vi "Render Read Pixels.vi"(6 "Pitch":i32 format="%.0x", 8 "error in":errorcluster, 9 "Format":u32 format="%.0x", 10 "Rectangle":T1, 11 "Renderer Pointer":u32 format="%.0x") -> (0 "error out":errorcluster, 2 "Pixels":i32[][](array[numeric]), 3 "Return":i32)   [LabVIEW 2021, in "LibSDL2.lvlib"]
uses:
  LibSDL2.lvlib
  DLL/SDL2.dll
  Controls/Rectangle.ctl
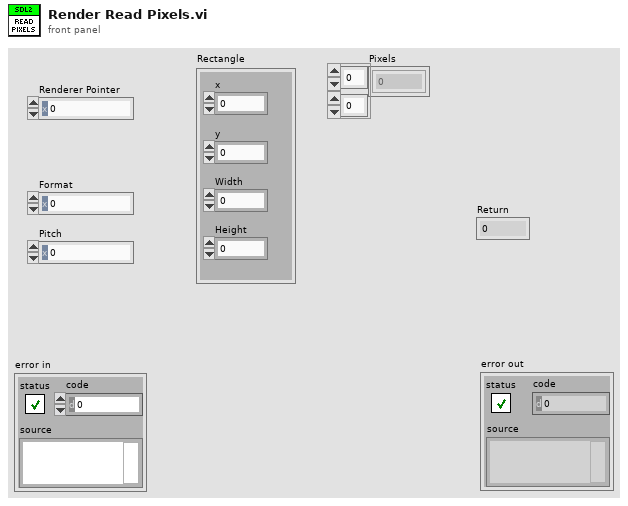
[diagram p1: front panel]
types:
  T1 = typedef "LibSDL2.lvlib/Rectangle.ctl" = cluster{"x":i32, "y":i32, "Width":i32, "Height":i32}
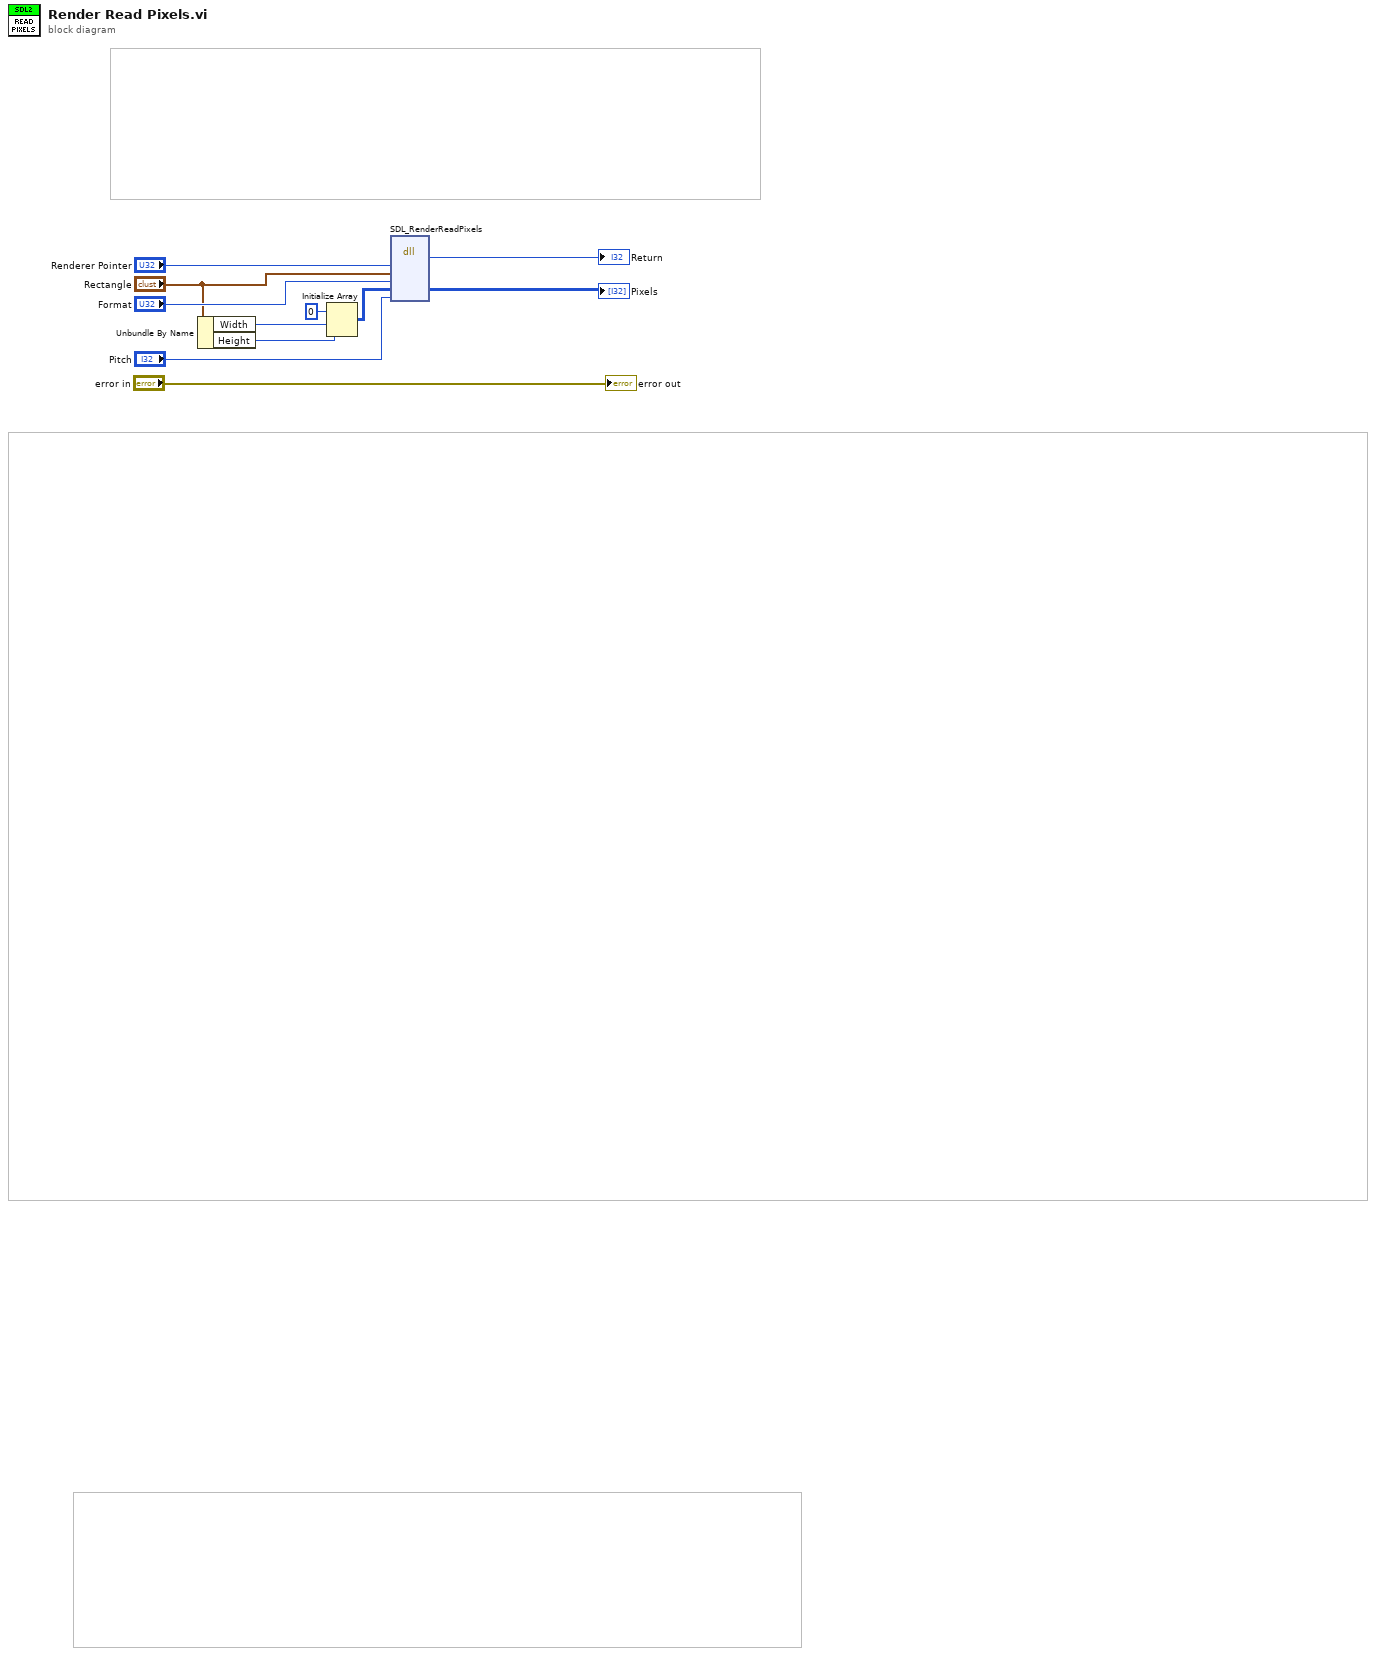
[diagram p0: block diagram]
diagram:
  n1 = Unbundle By Name("Rectangle") -> ("Width"=w2:i32, "Height"=w1:i32)
  n2 = Initialize Array(u32 0 ("element"), w2, w1) -> (w6:u32[][])
  n3 = dll-call lib="C:/dev/LabVIEW/LabSDL2/Source/Libraries/LibSDL2 Wrapper/DLL/SDL2.dll" fn="SDL_RenderReadPixels"("renderer"="Renderer Pointer", "rect"="Rectangle", "format"="Format", "pixels"=w6, "pitch"="Pitch") -> ("return type"=→"Return":i32, "pixels"=→"Pixels":i32[][])  [unwired: 7 in, 2 out]
  "error out" <- "error in"
